vi "Alerte Keller.vi"() -> ()   [LabVIEW 2022 SP3]
uses:
  Enum/Enum 2.ctl
  Variables globales/Variable glob alertes Keller.vi
  Variables globales/Variable glob Keller.vi
panel:
  out "Nb pages":u8
  in  "ajouter":bool
  in  "Groupes":T1(array[cluster])=[{"KELLER a surveiller :"=[0], "si pression > à ?"=1000.0, "Alerte"=FALSE, "N°"=0}] caption="Groupes alertes KELLER" {"si pression > à ?" min=1e-07 max=1000.0 step=1e-07}
  in  "OK":bool
  in  "Annuler":bool
  # "PARAMETRES POUR\nALERTE KELLER PAR ENVOI D'UN MAIL"
  # "Ce logiciel et les informations qu'il contient, sont la propriété de l’IAS et ne peuvent être diffusés sans l’autorisation de la Station d’étalonnage"
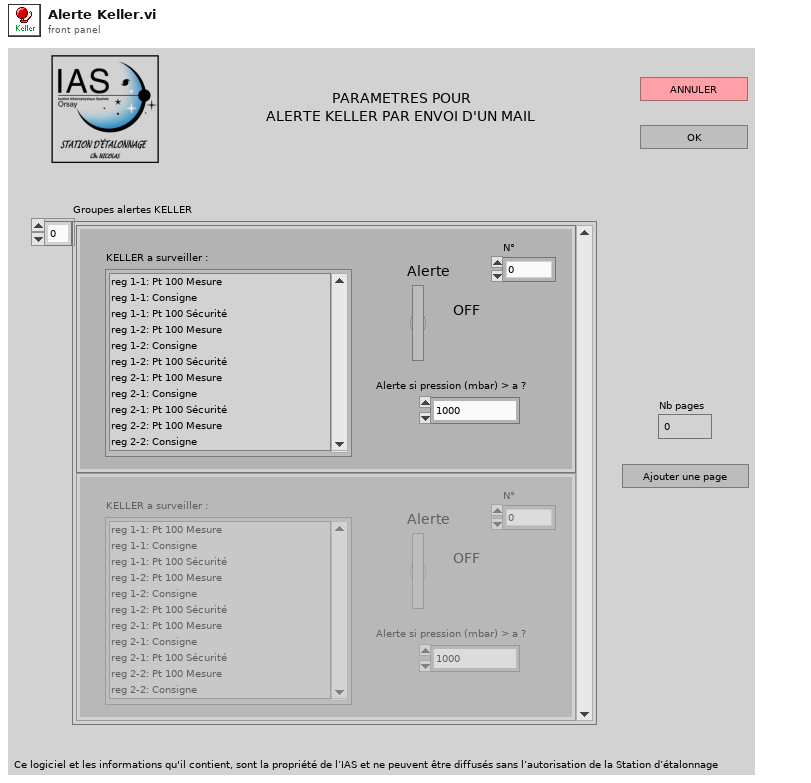
[diagram p1: front panel]
types:
  T1 = cluster{"KELLER a surveiller :":i32[], "si pression > à ?":dbl, "Alerte":bool, "N°":u16}[]
  T2 = typedef "Enum 2.ctl" = enum16{"init noms", "initialisation", "choix", "GO"}
  T3 = cluster{"Alerte Keller":bool, "valeur alerte Keller":dbl, "Défaut Keller":bool, "Indices Keller à controler":i16[], "N°":u16}[]
  T4 = cluster{"KELLER a surveiller :":i32[], "si pression > à ?":dbl, "Alerte":bool, "N°":u16}
  T5 = cluster{"Alerte Keller":bool, "valeur alerte Keller":dbl, "Défaut Keller":bool, "Indices Keller à controler":i16[], "N°":u16}
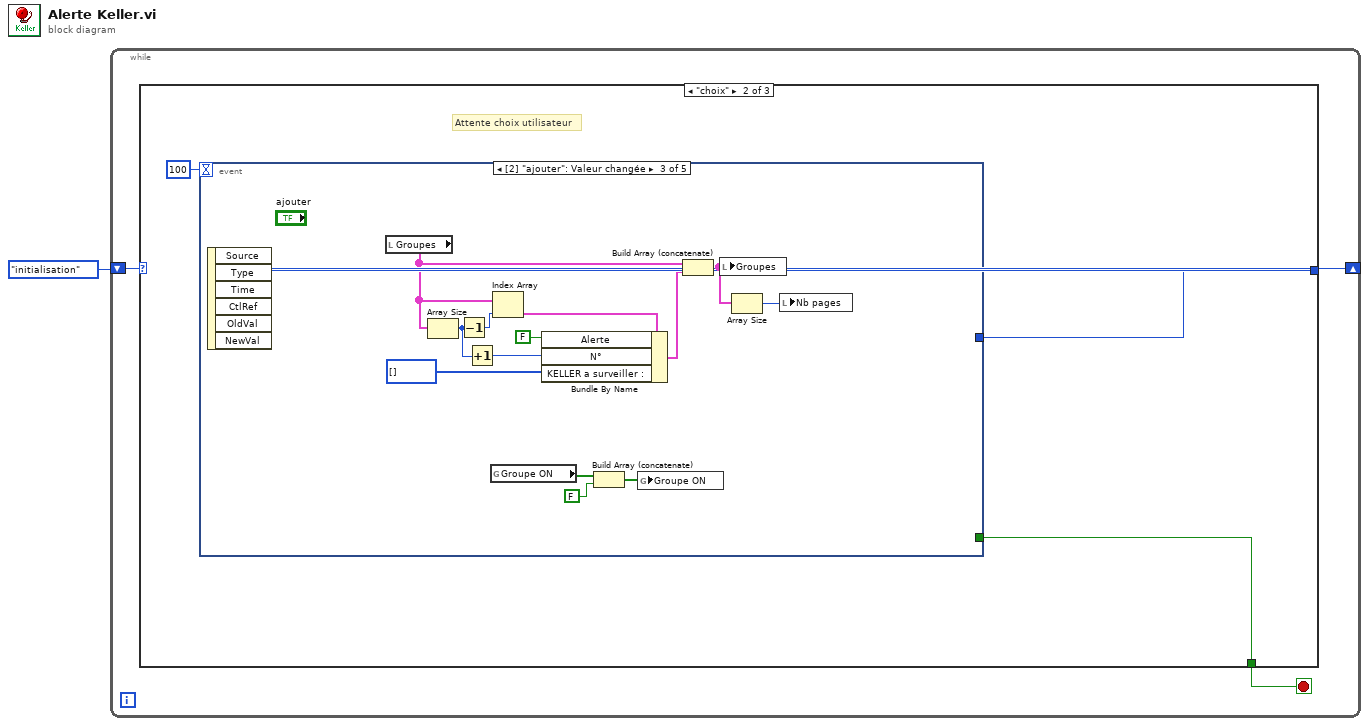
[diagram p0: block diagram]
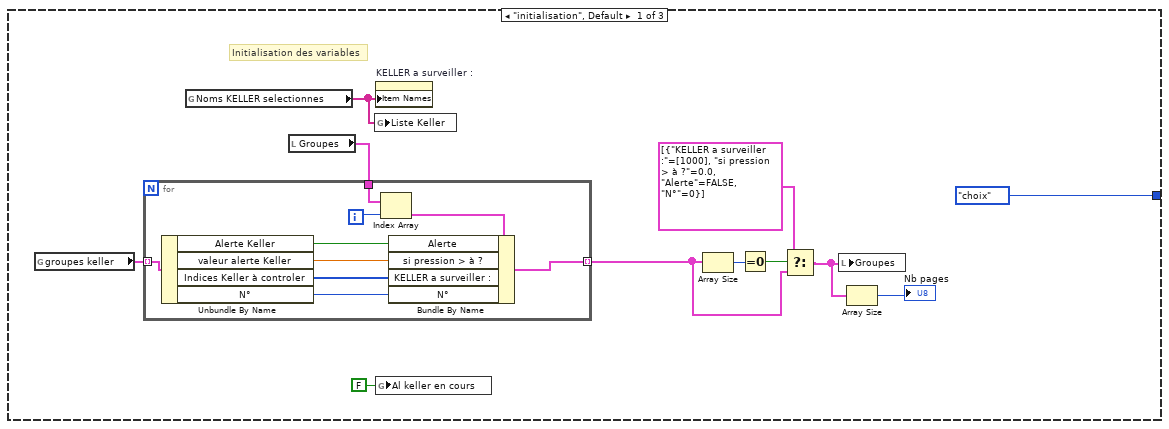
[diagram p2: hidden frame]
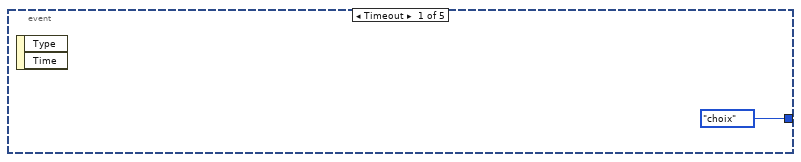
[diagram p3: hidden frame]
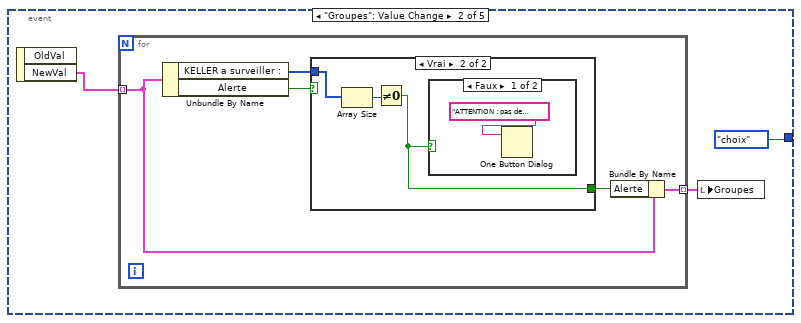
[diagram p4: hidden frame]
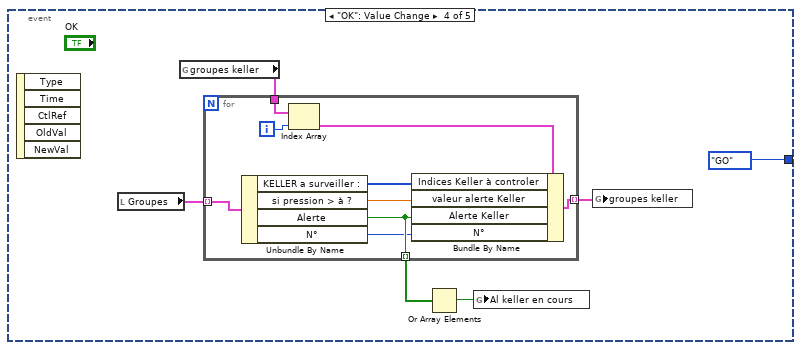
[diagram p7: hidden frame]
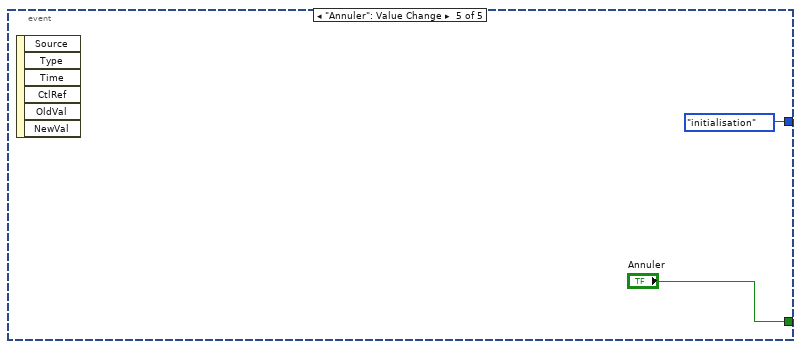
[diagram p8: hidden frame]
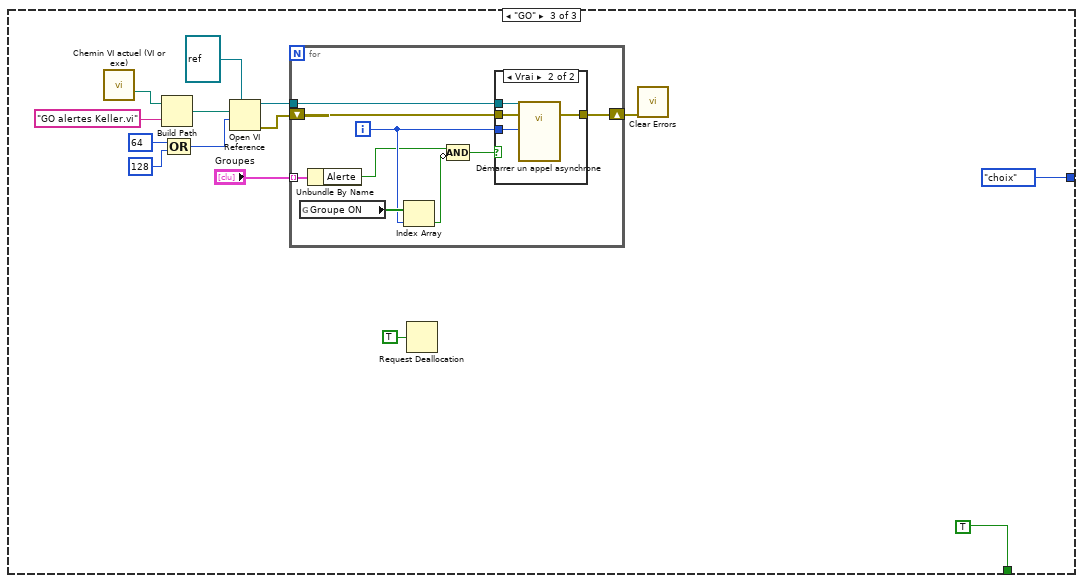
[diagram p9: hidden frame]
diagram:
  n1 = while {
    shift-right: [w3] -> _
    shift-left: Enum_2."initialisation" ("Énum") -> [w4]
    stop <- w2 stop-if-true
    n2 = case shown="\"choix\"" w4 {
      tunnel: [Enum_2."choix" ("Énum") w25 Enum_2."choix" ("Énum")] -> w3
      tunnel: [_ w26 TRUE] -> w2
      frame "initialisation", Default {
        # "Initialisation des variables"
        n3 = global read "Variable glob alertes Keller.vi" "groupes keller"() -> (w14:T3)
        n4 = global read "Variable glob Keller.vi" "Noms KELLER selectionnes"() -> (w11:string[])
        n5 = local read "Groupes"() -> (w13:T1)
        n6 = for {
          tunnel: w14 -> [w24] mode=indexing
          tunnel: w13 -> [w23]
          tunnel: [w18] -> w7 mode=indexing
          i -> [w17]
          n7 = Unbundle By Name(w24) -> ("Alerte Keller"=w19:bool, "valeur alerte Keller"=w21:dbl, "Indices Keller à controler"=w20:i16[], "N°"=w16:u16)
          n8 = Index Array(array=w23, index=w17) -> (element=w22:T4)
          n9 = Bundle By Name(cluster=w22, "Alerte"=w19, "si pression > à ?"=w21, "KELLER a surveiller :"=w20, "N°"=w16) -> (w18:T4)
        }
        n10 = global write "Variable glob alertes Keller.vi" "Liste Keller"(w11) -> ()
        n11 = property on="KELLER a surveiller :" class="LstDér (strict)"("Item Names"=w11) -> ()  [unwired: 2 in, 2 out]
        n12 = global write "Variable glob alertes Keller.vi" "Al keller en cours"(FALSE ("Al keller en cours")) -> ()
        n13 = Array Size(array=w7) -> (size(s)=w9:i32)
        n14 = Equal To 0?(x=w9) -> (x = 0?=w8:bool)
        n15 = Select(t=T1 [{"KELLER a surveiller :"=[1000], "si pression > à ?"=0.0, "Alerte"=FALSE, "N°"=0}] ("cas vrai"), s=w8, f=w7) -> (s? t:f=w6:T1)
        n16 = local write "Groupes"(w6) -> ()
        n17 = Array Size(array=w6) -> (size(s)=→"Nb pages":i32)
      }
      frame "choix" {
        # "Attente choix utilisateur"
        n18 = event shown="[2] \"ajouter\": Valeur changée" {
          selector: _ -> [_ _ _ _ _]
          dyn-events: _ -> [_ _ _ _ _]
          timeout: 100 -> [_ _ _ _ _]
          tunnel: [_ _ _ _ "Annuler"] -> w26
          tunnel: [Enum_2."choix" ("Énum") Enum_2."choix" ("Énum") _ Enum_2."GO" ("Énum") Enum_2."initialisation" ("Énum")] -> w25
          event Timeout {
            n19 = event-data() -> ()  [unwired: 1 in, 2 out]
          }
          event "Groupes": Value Change {
            n20 = event-data() -> ("NewVal"=w31:T1)  [unwired: 1 in, 1 out]
            n21 = for {
              tunnel: w31 -> [w35] mode=indexing
              tunnel: [w32] -> w30 mode=indexing
              n22 = Unbundle By Name(w35) -> ("KELLER a surveiller :"=w34:i32[], "Alerte"=w36:bool)
              n23 = case shown="Vrai" w36 {
                selector: w36 -> [w37 _]
                tunnel: w34 -> [_ w40]
                tunnel: [w37 w38] -> w33
                frame False {
                }
                frame True {
                  n24 = Array Size(array=w40) -> (size(s)=w39:i32)
                  n25 = Not Equal To 0?(x=w39) -> (x != 0?=w38:bool)
                  n26 = case shown="Faux" w38 {
                    frame False {
                      n27 = One Button Dialog(message="ATTENTION : pas de capteur choisi dans la liste") -> ()  [unwired: 1 in, 1 out]
                    }
                    frame True {
                    }
                  }
                }
              }
              n28 = Bundle By Name(cluster=w35, "Alerte"=w33) -> (w32:T4)
            }
            n29 = local write "Groupes"(w30) -> ()
          }
          event "ajouter": Value Change {
            n30 = event-data() -> ()  [unwired: 1 in, 6 out]
            n31 = local read "Groupes"() -> (w51:T1)
            n32 = Array Size(array=w51) -> (size(s)=w44:i32)
            n33 = Decrement(x=w44) -> (x-1=w50:i32)
            n34 = Increment(x=w44) -> (x+1=w43:i32)
            n35 = global read "Variable glob alertes Keller.vi" "Groupe ON"() -> (w47:bool[])
            n36 = Index Array(array=w51, index=w50) -> (element=w52:T4)
            n37 = Bundle By Name(cluster=w52, "Alerte"=FALSE, "N°"=w43, "KELLER a surveiller :"=i32[] []) -> (w54:T4)
            n38 = Build Array (concatenate)(w47, FALSE) -> (w45:bool[])
            n39 = global write "Variable glob alertes Keller.vi" "Groupe ON"(w45) -> ()
            n40 = Build Array (concatenate)(w51, w54) -> (w49:T1)
            n41 = local write "Groupes"(w49) -> ()
            n42 = Array Size(array=w49) -> (size(s)=w48:i32)
            n43 = local write "Nb pages"(w48) -> ()
          }
          event "OK": Value Change {
            n44 = event-data() -> ()  [unwired: 1 in, 5 out]
            n45 = local read "Groupes"() -> (w60:T1)
            n46 = global read "Variable glob alertes Keller.vi" "groupes keller"() -> (w59:T3)
            n47 = for {
              tunnel: w60 -> [w69] mode=indexing
              tunnel: w59 -> [w68]
              tunnel: [w63] -> w58 mode=indexing
              tunnel: [w62] -> w57 mode=indexing
              i -> [w67]
              n48 = Unbundle By Name(w69) -> ("KELLER a surveiller :"=w65:i32[], "si pression > à ?"=w64:dbl, "Alerte"=w62:bool, "N°"=w61:u16)
              n49 = Index Array(array=w68, index=w67) -> (element=w66:T5)
              n50 = Bundle By Name(cluster=w66, "Indices Keller à controler"=w65, "valeur alerte Keller"=w64, "Alerte Keller"=w62, "N°"=w61) -> (w63:T5)
            }
            n51 = Or Array Elements(Boolean array=w57) -> (logical OR=w56:bool)
            n52 = global write "Variable glob alertes Keller.vi" "Al keller en cours"(w56) -> ()
            n53 = global write "Variable glob alertes Keller.vi" "groupes keller"(w58) -> ()
          }
          event "Annuler": Value Change {
            n54 = event-data() -> ()  [unwired: 1 in, 6 out]
          }
        }
      }
      frame "GO" {
        n55 = call "Chemin VI actuel (VI or exe).vi"() -> ("VI or executable installation directory"=w79:path)  [unwired: 14 in, 1 out]
        n56 = Build Path(base path=w79, name or relative path="GO alertes Keller.vi" ("nom ou chemin relatif")) -> (appended path=w74:path)
        n57 = Compound Arithmetic op=OR(64 ("options"), 128 ("options")) -> (w78:i32)
        n58 = Open VI Reference(type specifier VI Refnum (for type only)=refnum<vi> refnum ("spécificateur de type du refnum de VI (pour type seulement)"), vi path=w74, options=w78) -> (vi reference=w80:refnum<vi>, error out=w81:errorcluster)  [unwired: 3 in]
        n59 = for {
          shift-right: [w93] -> w83
          shift-left: w81 -> [w94]
          tunnel: w80 -> [w92]
          tunnel: "Groupes" -> [w91] mode=indexing
          i -> [w89]
          n60 = global read "Variable glob alertes Keller.vi" "Groupe ON"() -> (w90:bool[])
          n61 = Unbundle By Name(w91) -> ("Alerte"=w88:bool)
          n62 = Index Array(array=w90, index=w89) -> (element=w87:bool)
          n63 = Compound Arithmetic op=AND ("Opérateur arithmétique")(w88, invert w87) -> (w86:bool)
          n64 = case shown="Vrai" w86 {
            tunnel: w94 -> [w95 w99]
            tunnel: [w95 w98] -> w93
            tunnel: w92 -> [_ w97]
            tunnel: w89 -> [_ w96]
            frame False {
            }
            frame True {
              n65 = call-by-ref "Démarrer un appel asynchrone"(reference=w97, error in=w99, "Numéro"=w96) -> (error out=w98:errorcluster)  [unwired: 5 in, 1 out]
            }
          }
        }
        n66 = Request Deallocation(TRUE ("flag")) -> ()
        n67 = call <vilib>:"Clear Errors.vi"("error in (no error)"=w83) -> ()  [unwired: 5 in, 2 out]
      }
    }
  }
